vi "piano UI.vi"() -> ()   [LabVIEW 2020]
uses:
  midi-ui/midi-ui.lvclass
  midi-file/Note Value.ctl
  midi-file/midi-file.lvclass
  <vilib>/Analysis/NI_AAL_Geometry.lvlib
  <vilib>/Analysis/geometry.llb/Point in Polygon Position.ctl
  midi/midi.lvclass
  <vilib>/Analysis/geometry.llb/Point in Polygon (Scalar).vi
panel:
  out "Data2":i32
  out "Data1":i32
  out "Status":i32
  out "Sustain":bool
  in  "Note Off":bool
  in  "Note On":bool
  in  "Note Value":T1
  out "2D Picture":picture
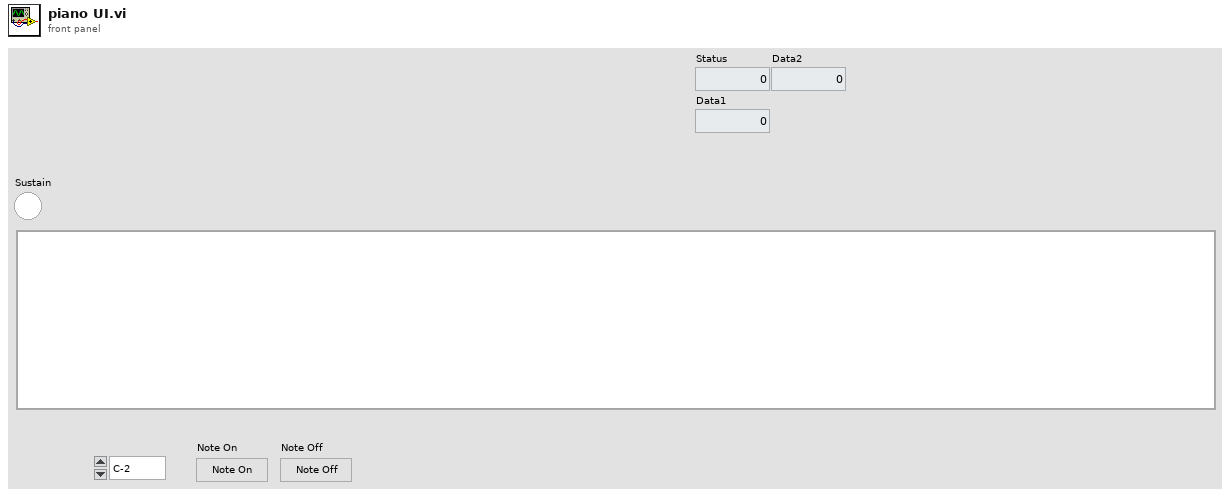
[diagram p1: front panel]
types:
  T1 = typedef "midi-file.lvclass/Note Value.ctl" = enum8{"C-2", "C#-2", "D-2", "D#-2", "E-2", "F-2", "F#-2", "G-2", "G#-2", "A-2", "A#-2", "B-2", "C-1", "C#-1", "D-1", "D#-1", "E-1", "F-1", "F#-1", "G-1", "G#-1", "A-1", "A#-1", "B-1", "C0", "C#0", "D0", "D#0", "E0", "F0", "F#0", "G0", "G#0", "A0", "A#0", "B0", "C1", "C#1", "D1", "D#1", "E1", "F1", "F#1", "G1", "G#1", "A1", "A#1", "B1", "C2", "C#2", "D2", "D#2", "E2", "F2", "F#2", "G2", "G#2", "A2", "A#2", "B2", "C3", "C#3", "D3", "D#3", "E3", "F3", "F#3", "G3", "G#3", "A3", "A#3", "B3", "C4", "C#4", "D4", "D#4", "E4", "F4", "F#4", "G4", "G#4", "A4", "A#4", "B4", "C5", "C#5", "D5", "D#5", "E5", "F5", "F#5", "G5", "G#5", "A5", "A#5", "B5", "C6", "C#6", "D6", "D#6", "E6", "F6", "F#6", "G6", "G#6", "A6", "A#6", "B6", "C7", "C#7", "D7", "D#7", "E7", "F7", "F#7", "G7", "G#7", "A7", "A#7", "B7", "C8", "C#8", "D8", "D#8", "E8", "F8", "F#8", "G"}
  T2 = cluster{"Width":u16, "Style":enum32{"Solid", "Dash", "Dot", "DashDot", "DashDotDot"}}
  T3 = typedef "LVPoint32TypeDef.ctl" = cluster{"Horizontal":i32, "Vertical":i32}
  T4 = typedef "NI_AAL_Geometry.lvlib/Point in Polygon Position.ctl" = u16
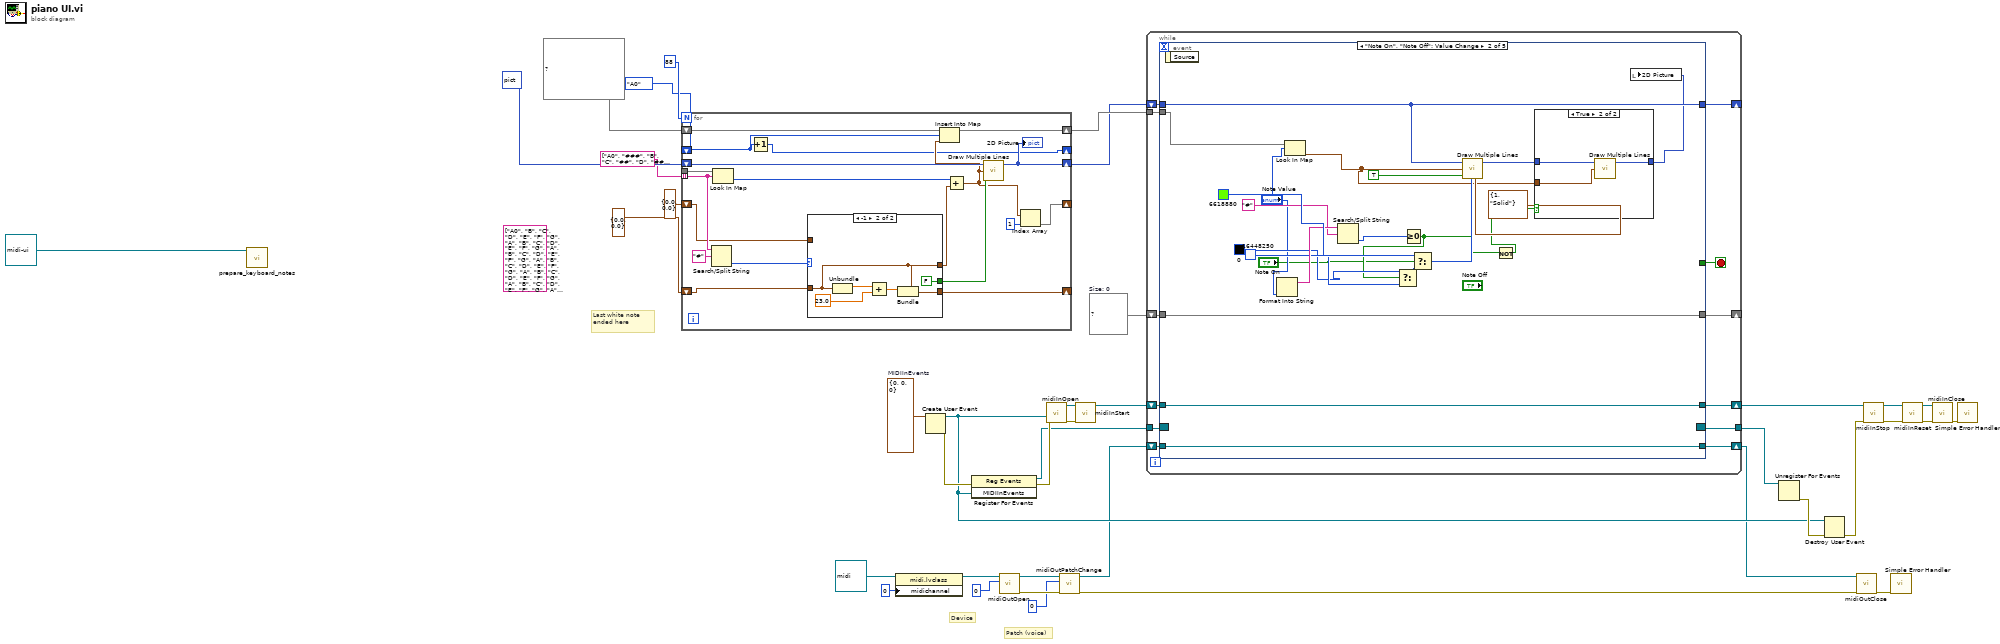
[diagram p0: block diagram]
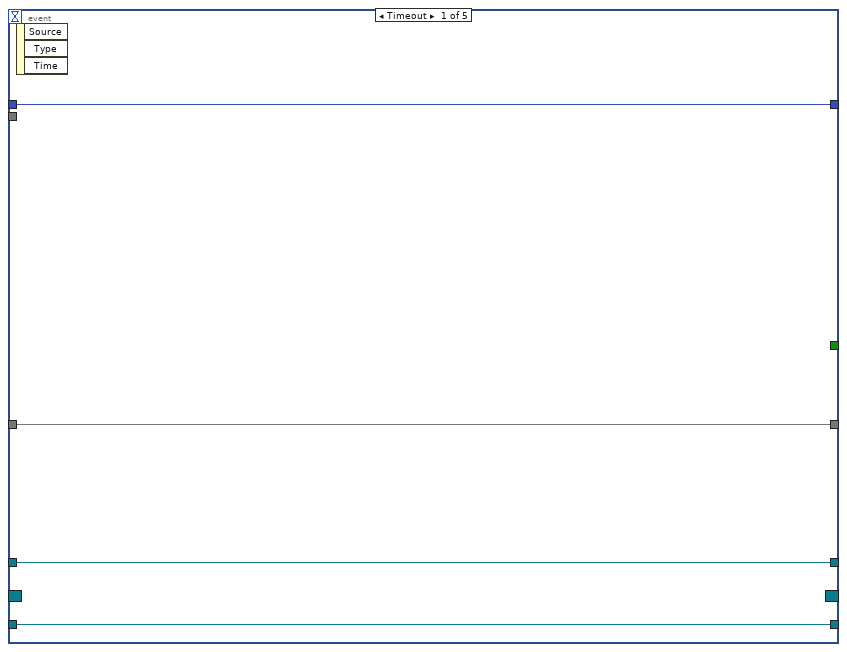
[diagram p2: hidden frame]
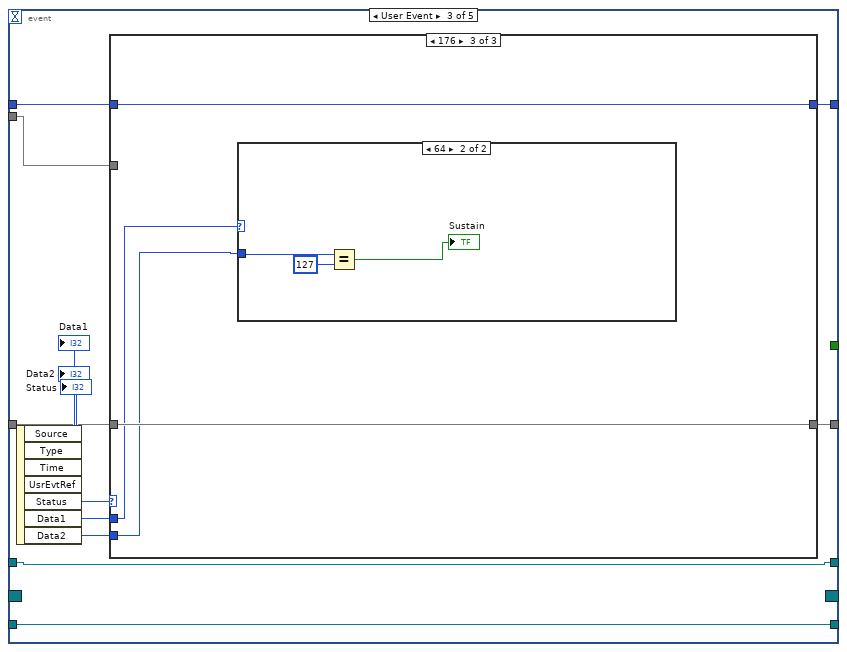
[diagram p4: hidden frame]
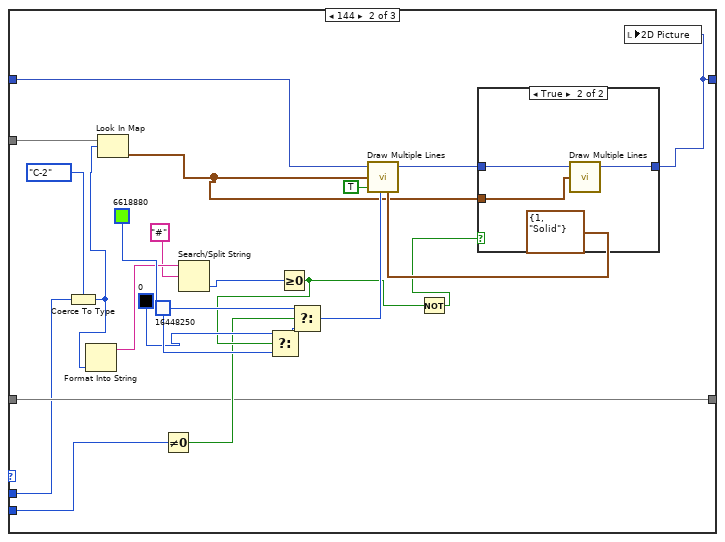
[diagram p6: hidden frame]
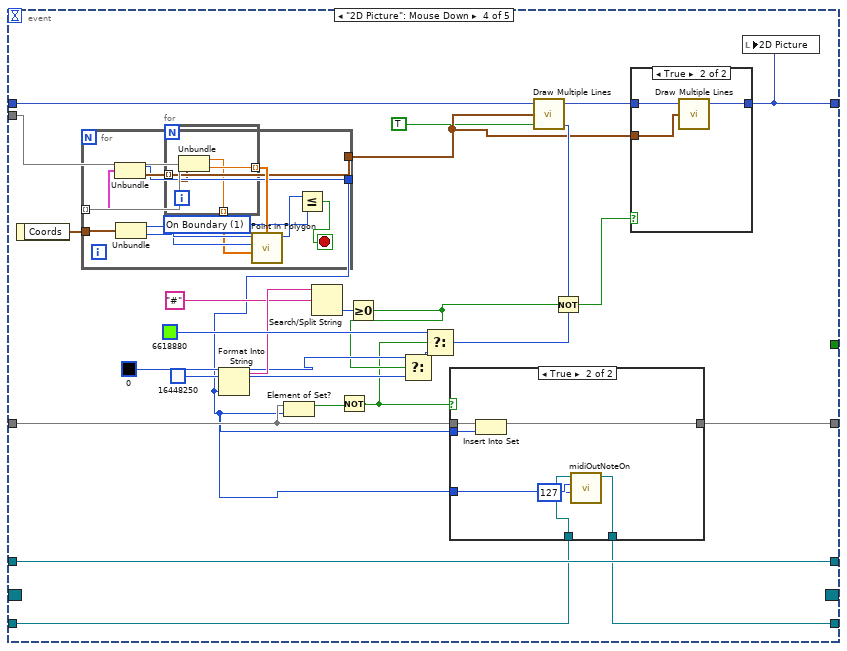
[diagram p9: hidden frame]
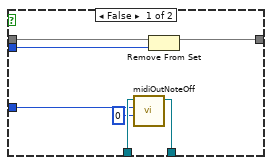
[diagram p10: hidden frame]
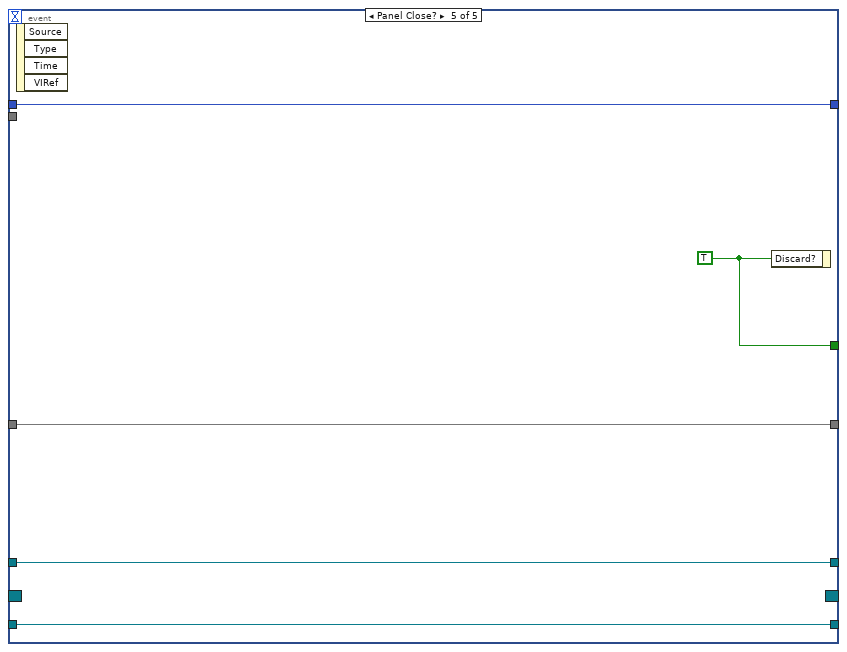
[diagram p12: hidden frame]
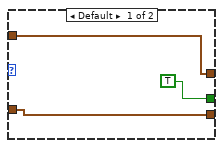
[diagram p13: hidden frame]
diagram:
  w25 = cluster{"Status":i32, "Data1":i32, "Data2":i32} {"Status"=0, "Data1"=0, "Data2"=0}  # MIDIInEvents
  w30 = set{T1} {}  # Size: 0
  (unwired) string[] ["A0", "B", "C", "D", "E", "F", "G", "A", "B", "C", "D", "E", "F", "G", "A", "B", "C", "D", "E", "F", "G", "A", "B", "C", "D", "E", "F", "G", "A", "B", "C", "D", "E", "F", "G", "A", "B", "C", "D", "E", "F", "G", "A", "B", "C", "D", "E", "F", "G", "A", "B", "C8"] ("array")
  # "Patch (voice)"
  # "Device"
  # "Last white note ended here"
  n1 = call "prepare_keyboard_notes.vi"("midi-ui in"=refnum<class "midi-ui.lvclass"> refnum) -> ()  [unwired: 9 in, 2 out]
  n2 = for {
    N: 88 -> [_]
    tunnel: [w57] -> w39
    shift-right: [w58] -> w31
    shift-left: picture data[5B] ("picture") -> [w59]
    tunnel: string[] ["A0", "###", "B", "C", "##", "D", "##", "E", "F", "###", "G", "###", "A", "###", "B", "C", "##", "D", "##", "E", "F", "###", "G", "###", "A", "###", "B", "C", "##", "D", "##", "E", "F", "###", "G", "###", "A", "###", "B", "C", "##", "D", "##", "E", "F", "###", "G", "###", "A", "###", "B", "C", "##", "D", "##", "E", "F", "###", "G", "###", "A", "###", "B", "C", "##", "D", "##", "E", "F", "###", "G", "###", "A", "###", "B", "C", "##", "D", "##", "E", "F", "###", "G", "###", "A", "###", "B", "C8", "D", "##", "E", "F", "###", "G", "###", "A", "###", "B", "C", "##", "D", "##", "E", "F", "###", "G", "###", "A", "###", "B", "C", "##", "D", "##", "E", "F", "###", "G", "### ", ""] ("array") -> [w55] mode=indexing
    shift-right: [w52] -> _
    shift-left: cluster{"x":dbl, "y":dbl} {"x"=0.0, "y"=0.0} ("coordinate") -> [w51]
    shift-right: [w47] -> _
    shift-left: cluster{"x":dbl, "y":dbl} {"x"=0.0, "y"=0.0} ("coordinate") -> [w49]
    shift-right: [w43] -> w32
    shift-left: map{T1, cluster{"x":dbl, "y":dbl}[]} {} ("map in") -> [w44]
    shift-right: [w41] -> _
    shift-left: Note_Value."A0" ("Note Value") -> [w42]
    n3 = Search/Split String(string=w55, search string/char (-)="#") -> (offset of match=w53:i32)  [unwired: 1 in, 2 out]
    n4 = Look In Map(map=w57, key=w55) -> (value=w56:i32)  [unwired: 1 in, 1 out]
    n5 = Increment(x=w42) -> (x+1=w41:T1)
    n6 = case shown="-1" w53 {
      tunnel: w51 -> [w62 w64]
      tunnel: [w62 w65] -> w52
      tunnel: [w61 w64] -> w50
      tunnel: w49 -> [w61 _]
      tunnel: [TRUE FALSE] -> w46
      frame Default {
      }
      frame -1 {
        n7 = Unbundle(w64) -> ("x"=w68:dbl)  [unwired: 1 out]
        n8 = Add(x=w68, y=23.0) -> (x+y=w66:dbl)
        n9 = Bundle(cluster=w64, "x"=w66) -> (w65:cluster{"x":dbl, "y":dbl})  [unwired: 1 in]
      }
    }
    n10 = Add(x=w56, y=w50) -> (x+y=w45:cluster{"x":dbl, "y":dbl})
    n11 = Insert Into Map(map in=w44, key=w42, value=w45) -> (map out=w43:map{T1, cluster{"x":dbl, "y":dbl}[]})  [unwired: 2 out]
    n12 = call <vilib>:"Draw Multiple Lines.vi"("picture"=w59, "line endpoints"=w45, "fill?(F)"=w46) -> ("new picture"=w58:picture)  [unwired: 6 in]
    "2D Picture" <- w58
    n13 = Index Array(array=w45, index=1) -> (element=w47)
  }
  n14 = property class="midi.lvclass"(reference=refnum<class "midi.lvclass"> refnum ("midi in"), "midichannel"=u64 0) -> (reference out=w5:refnum<class "midi.lvclass">)  [unwired: 1 in, 1 out]
  n15 = Create User Event(user event datatype=w25) -> (user event=w13:refnum<user-event>, error out=w27:errorcluster)  [unwired: 1 in]
  n16 = register-events(error in=w27, w13) -> (reference out=w15:refnum<event-registration>, error out=w28:errorcluster)  [unwired: 1 in]
  n17 = call "midiOutOpen.vi"("DeviceID"=u32 0, "midi in"=w5) -> ("error out"=w9:errorcluster, "midi out"=w10:refnum<class "midi.lvclass">)  [unwired: 8 in]
  n18 = call "midiInOpen.vi"("error in"=w28, "MidiDataEvents"=w13) -> ("error out"=w18:errorcluster, "midi out"=w19:refnum<class "midi.lvclass">)  [unwired: 8 in]
  n19 = call "midiOutPatchChange.vi"("error in"=w9, "Patch"=u32 0, "midi in"=w10) -> ("error out"=w2:errorcluster, "midi out"=w4:refnum<class "midi.lvclass">)  [unwired: 7 in]
  n20 = call "midiInStart.vi"("error in"=w18, "midi in"=w19) -> ("midi out"=w17:refnum<class "midi.lvclass">)  [unwired: 8 in, 1 out]
  n21 = while {
    tunnel: w32 -> [w80]
    shift-right: [w76] -> _
    shift-left: w30 -> [w77]
    shift-right: [w75] -> _
    shift-left: w31 -> [w79]
    shift-right: [w73] -> w16
    shift-left: w17 -> [w74]
    tunnel: w15 -> [w72]
    tunnel: [w71] -> w14
    shift-right: [w69] -> w3
    shift-left: w4 -> [w70]
    stop <- w78 stop-if-true
    n22 = event shown="[1] \"Note On\", \"Note Off\": Value Change" {
      selector: w72 -> [_ _ _ _ _]
      dyn-events: [_ _ _ _ _] -> w71
      timeout: _ -> [_ _ _ _ _]
      tunnel: w80 -> [_ w106 w120 w170 _]
      tunnel: w79 -> [w83 w105 w119 w181 w216]
      tunnel: [_ _ _ _ w218] -> w78
      tunnel: w77 -> [w84 w89 w113 w165 w217]
      tunnel: [w84 w89 w114 w164 w217] -> w76
      tunnel: [w83 w105 w112 w163 w216] -> w75
      tunnel: w74 -> [w82 w86 w115 w160 w215]
      tunnel: [w82 w86 w115 w160 w215] -> w73
      tunnel: w70 -> [w81 w85 w111 w159 w214]
      tunnel: [w81 w85 w111 w158 w214] -> w69
      event Timeout {
        n23 = event-data() -> ()  [unwired: 1 in, 3 out]
      }
      event "Note On", "Note Off": Value Change {
        n24 = event-data() -> ()  [unwired: 1 in, 1 out]
        n25 = Format Into String("Note Value") -> (resulting string=w102:string)  [unwired: 3 in, 1 out]
        n26 = Look In Map(map=w106, key="Note Value") -> (value=w92:cluster{"x":dbl, "y":dbl}[])  [unwired: 1 in, 1 out]
        n27 = Search/Split String(string=w102, search string/char (-)="#") -> (offset of match=w100:i32)  [unwired: 1 in, 2 out]
        n28 = Greater Or Equal To 0?(x=w100) -> (x >= 0?=w91:bool)
        n29 = Select(t=u32 0 ("color(black)"), s=w91, f=u32 16448250 ("color(black)")) -> (s? t:f=w97:u32)
        n30 = Select(t=u32 6618880 ("color(black)"), s="Note On", f=w97) -> (s? t:f=w103:u32)
        n31 = call <vilib>:"Draw Multiple Lines.vi"("picture"=w105, "line endpoints"=w92, "fill?(F)"=TRUE, "color(black)"=w103, "pen"=T2 {"Width"=1, "Style"=enum."Solid"}) -> ("new picture"=w93:picture)  [unwired: 4 in]
        n32 = Not(x=w91) -> (.not. x?=w90:bool)
        n33 = case shown="True" w90 {
          tunnel: [w107 w109] -> w94
          tunnel: w93 -> [w107 w110]
          tunnel: w92 -> [_ w108]
          frame False {
          }
          frame True {
            n34 = call <vilib>:"Draw Multiple Lines.vi"("picture"=w110, "line endpoints"=w108) -> ("new picture"=w109:picture)  [unwired: 7 in]
          }
        }
        n35 = local write "2D Picture"(w94) -> ()
      }
      event User Event {
        n36 = event-data() -> ("Status"=w116:i32, "Data1"=w118:i32, "Data2"=w117:i32)  [unwired: 1 in, 4 out]
        "Status" <- w116
        "Data1" <- w118
        "Data2" <- w117
        n37 = case shown="176" w116 {
          tunnel: w120 -> [_ w145 _]
          tunnel: w119 -> [w121 w144 w152]
          tunnel: w118 -> [_ w124 w151]
          tunnel: w117 -> [_ w128 w150]
          tunnel: [w122 w127 w153] -> w114
          tunnel: w113 -> [w122 w127 w153]
          tunnel: [w121 w126 w152] -> w112
          frame 0, Default {
          }
          frame 144 {
            n38 = Coerce To Type(0:w124, 1:Note_Value."C-2" ("key")) -> (2:w123:T1)
            n39 = Format Into String(w123) -> (resulting string=w141:string)  [unwired: 3 in, 1 out]
            n40 = Look In Map(map=w145, key=w123) -> (value=w133:cluster{"x":dbl, "y":dbl}[])  [unwired: 1 in, 1 out]
            n41 = Not Equal To 0?(x=w128) -> (x != 0?=w129:bool)
            n42 = Search/Split String(string=w141, search string/char (-)="#") -> (offset of match=w139:i32)  [unwired: 1 in, 2 out]
            n43 = Greater Or Equal To 0?(x=w139) -> (x >= 0?=w132:bool)
            n44 = Select(t=u32 0 ("color(black)"), s=w132, f=u32 16448250 ("color(black)")) -> (s? t:f=w136:u32)
            n45 = Select(t=u32 6618880 ("color(black)"), s=w129, f=w136) -> (s? t:f=w142:u32)
            n46 = call <vilib>:"Draw Multiple Lines.vi"("picture"=w144, "line endpoints"=w133, "fill?(F)"=TRUE, "color(black)"=w142, "pen"=T2 {"Width"=1, "Style"=enum."Solid"}) -> ("new picture"=w134:picture)  [unwired: 4 in]
            n47 = Not(x=w132) -> (.not. x?=w131:bool)
            n48 = case shown="True" w131 {
              tunnel: [w146 w148] -> w126
              tunnel: w134 -> [w146 w149]
              tunnel: w133 -> [_ w147]
              frame False {
              }
              frame True {
                n49 = call <vilib>:"Draw Multiple Lines.vi"("picture"=w149, "line endpoints"=w147) -> ("new picture"=w148:picture)  [unwired: 7 in]
              }
            }
            n50 = local write "2D Picture"(w126) -> ()
          }
          frame 176 {
            n51 = case shown="64" w151 {
              tunnel: w150 -> [_ w156]
              frame 0, Default {
              }
              frame 64 {
                n52 = Equal?(x=w156, y=127) -> (x = y?=→"Sustain":bool)
              }
            }
          }
        }
      }
      event "2D Picture": Mouse Down {
        n53 = event-data() -> ("Coords"=w169:T3)  [unwired: 1 in]
        n54 = for {
          tunnel: w170 -> [w203] mode=indexing
          tunnel: w169 -> [w206]
          tunnel: [w197] -> w168
          tunnel: [w196] -> w157
          stop <- w198 stop-if-true
          w199 = T4 1 items=["Inside", "On Boundary", "Outside"] ("y")
          n55 = Unbundle(w203) -> ("Note Value"=w196:T1, w197:cluster{"x":dbl, "y":dbl}[])
          n56 = Unbundle(w206) -> ("Horizontal"=w205:i32, "Vertical"=w204:i32)
          n57 = for {
            tunnel: w197 -> [w209] mode=indexing
            tunnel: [w208] -> w201 mode=indexing
            tunnel: [w207] -> w202 mode=indexing
            n58 = Unbundle(w209) -> ("x"=w207:dbl, "y"=w208:dbl)
          }
          n59 = call-poly <vilib>:"Point in Polygon.vi"("Polygon Y"=w201, "Polygon X"=w202, "y"=w204, "x"=w205) -> ("position"=w200:T4)  [unwired: 6 in, 1 out]
          n60 = Less Or Equal?(x=w200, y=w199) -> (x <= y?=w198:bool)
        }
        n61 = Format Into String(w157) -> (resulting string=w178:string)  [unwired: 3 in, 1 out]
        n62 = Element of Set?(10:w157, 11:w165) -> (3:w166:bool)
        n63 = Search/Split String(string=w178, search string/char (-)="#") -> (offset of match=w176:i32)  [unwired: 1 in, 2 out]
        n64 = Not(x=w166) -> (.not. x?=w162:bool)
        n65 = Greater Or Equal To 0?(x=w176) -> (x >= 0?=w167:bool)
        n66 = Select(t=u32 0 ("color(black)"), s=w167, f=u32 16448250 ("color(black)")) -> (s? t:f=w173:u32)
        n67 = Select(t=u32 6618880 ("color(black)"), s=w162, f=w173) -> (s? t:f=w179:u32)
        n68 = case shown="True" w162 {
          tunnel: w165 -> [w188 w195]
          tunnel: [w186 w194] -> w164
          tunnel: w157 -> [w187 w193]
          tunnel: w159 -> [w185 w192]
          tunnel: [w184 w191] -> w158
          tunnel: w157 -> [w183 w190]
          frame False {
            n69 = call "midiOutNoteOff.vi"("Velocity (0-127)"=0, "Note (0-127)"=w183, "midi in"=w185) -> ("midi out"=w184:refnum<class "midi.lvclass">)  [unwired: 7 in, 1 out]
            n70 = Remove From Set(10:w187, 11:w188) -> (3:w186:set{T1})  [unwired: 1 out]
          }
          frame True {
            n71 = Insert Into Set(10:w193, 11:w195) -> (3:w194:set{T1})  [unwired: 1 out]
            n72 = call "midiOutNoteOn.vi"("Velocity (0-127)"=127, "Note (0-127)"=w190, "midi in"=w192) -> ("midi out"=w191:refnum<class "midi.lvclass">)  [unwired: 7 in, 1 out]
          }
        }
        n73 = call <vilib>:"Draw Multiple Lines.vi"("picture"=w181, "line endpoints"=w168, "fill?(F)"=TRUE, "color(black)"=w179) -> ("new picture"=w172:picture)  [unwired: 5 in]
        n74 = Not(x=w167) -> (.not. x?=w171:bool)
        n75 = case shown="True" w171 {
          tunnel: [w210 w212] -> w163
          tunnel: w172 -> [w210 w213]
          tunnel: w168 -> [_ w211]
          frame False {
          }
          frame True {
            n76 = call <vilib>:"Draw Multiple Lines.vi"("picture"=w213, "line endpoints"=w211) -> ("new picture"=w212:picture)  [unwired: 7 in]
          }
        }
        n77 = local write "2D Picture"(w163) -> ()
      }
      event Panel Close? {
        w218 = TRUE
        n78 = event-data() -> ()  [unwired: 1 in, 4 out]
        n79 = event-data("Discard?"=w218) -> ()  [unwired: 1 in, 1 out]
      }
    }
  }
  n80 = Unregister For Events(event registration refnum=w14) -> (error out=w29:errorcluster)  [unwired: 1 in]
  n81 = Destroy User Event(user event=w13, error in=w29) -> (error out=w24:errorcluster)
  n82 = call "midiOutClose.vi"("error in"=w2, "midi in"=w3) -> ("error out"=w12:errorcluster)  [unwired: 8 in, 1 out]
  n83 = call "midiInStop.vi"("error in"=w24, "midi in"=w16) -> ("error out"=w23:errorcluster, "midi out"=w22:refnum<class "midi.lvclass">)  [unwired: 8 in]
  n84 = call <vilib>:"Simple Error Handler.vi"("error in (no error)"=w12) -> ()  [unwired: 4 in, 5 out]
  n85 = call "midiInReset.vi"("error in"=w23, "midi in"=w22) -> ("error out"=w21:errorcluster, "midi out"=w20:refnum<class "midi.lvclass">)  [unwired: 8 in]
  n86 = call "midiInClose.vi"("error in"=w21, "midi in"=w20) -> ("error out"=w26:errorcluster)  [unwired: 8 in, 1 out]
  n87 = call <vilib>:"Simple Error Handler.vi"("error in (no error)"=w26) -> ()  [unwired: 4 in, 5 out]
